vi "UE_Percent_Drop.vi"(2 "final":dbl, 3 "initial":dbl) -> (0 "valid":bool, 1 "percent_drop":dbl)   [LabVIEW 2026]
doc: "INTENT: Compute 100 times (initial minus final) divided by initial only for initial > 0. INPUTS: initial (double), final (double). OUTPUTS: percent_drop (double), valid (bool). DESIGN CONSTRAINT: Invalid initial produces 0 percent and valid=false; caller must reject invalid result. REQUIREMENTS: SRS-F-008. No physical hardware side effects. Acceptance requires native LabVIEW compilation and behavioral testing."
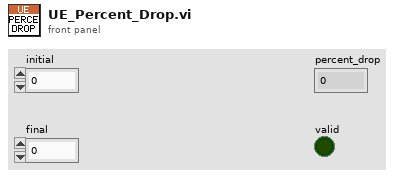
[diagram p1: front panel]
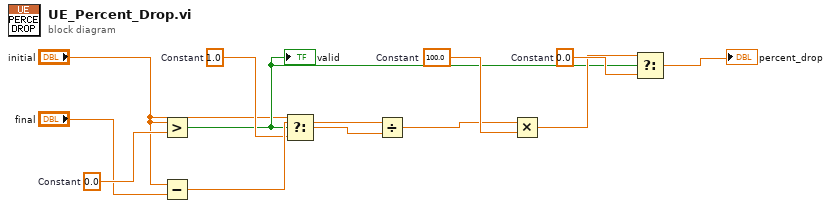
[diagram p0: block diagram]
diagram:
  w11 = 0.0  # Constant
  w9 = 100.0  # Constant
  w5 = 1.0  # Constant
  w3 = 0.0  # Constant
  n1 = Greater?(x="initial", y=w3) -> (0:w4:bool)
  "valid" <- w4
  n2 = Subtract(x="initial", y="final") -> (x-y=w7:dbl)
  n3 = Select(t="initial", s=w4, f=w5) -> (s? t:f=w6:dbl)
  n4 = Divide(x=w7, y=w6) -> (x/y=w8:dbl)
  n5 = Multiply(x=w8, y=w9) -> (x*y=w10:dbl)
  n6 = Select(t=w10, s=w4, f=w11) -> (s? t:f=→"percent_drop":dbl)
